vi "http.post.vi"(6 "specific headers in":cluster{"header":string, "Value":string}[](array[cluster]), 7 "Content Type":string="application/json", 8 "error in":errorcluster, 9 "Request body":string, 10 "Path":string, 11 "Nominal Client in":refnum<class "Nominal Client.lvclass">) -> (0 "error out":errorcluster, 2 "Response":string, 3 "Nominal Client out":refnum<class "Nominal Client.lvclass">)   [LabVIEW 2020, in "Nominal Client.lvclass"]
uses:
  Nominal Client.lvclass
  Nominal Client.lvclass/Nominal Client.ctl
  trace.calling_method.vi
  error.vi/859f8e04-e495-489b-b5b4-7ac163f56130.vi
  <vilib>/JDP Science/JDP Science Common Utilities/Trim Whitespace__JDP.vi
  <vilib>/AdvancedString/1D String Array to Delimited String.vi
  api_token.get.vi
  <vilib>/Utility/libraryn.llb/Get File Extension.vi
  log_file.write.vi
  <vilib>/JDP Science/JSONtext/Get all Object Items.vi
  <vilib>/Utility/error.llb/Error Cluster From Error Code.vi
  <vilib>/JDP Science/JSONtext/JSON text to Variant.vi
  <vilib>/JDP Science/JSONtext/LVClass Serializer/JSONtext LVClass Serializer.lvclass
  submodules/reqwest-labview/lv-src/reqwest/reqwest.lvclass
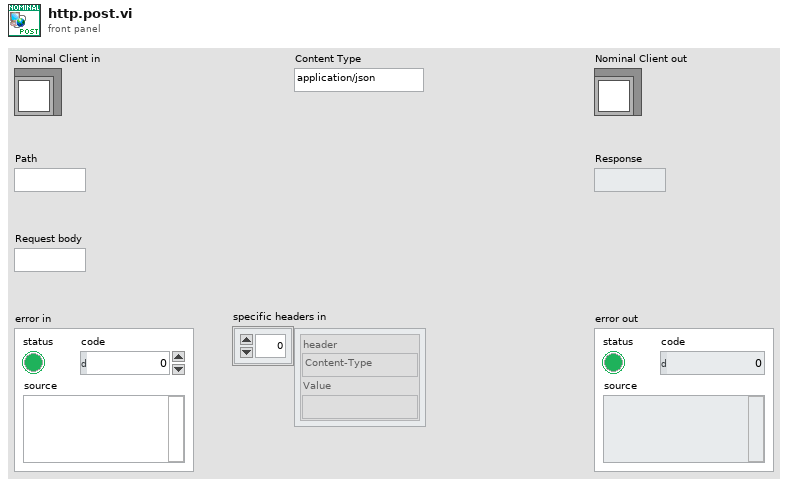
[diagram p1: front panel]
types:
  T1 = typedef "Nominal Client.lvclass/private_data.ctl" = cluster{"API Token":string, "workspace":refnum<class "workspace.lvclass">, "Available Workspaces":refnum<class "workspace.lvclass">[], "reqwest":refnum<class "reqwest.lvclass">}
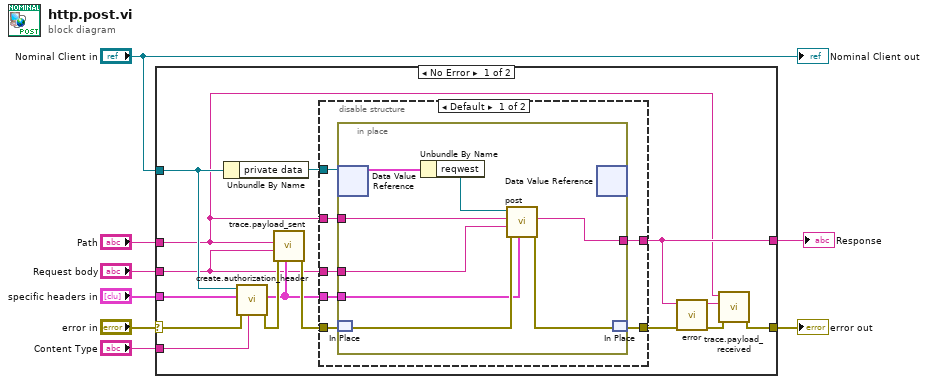
[diagram p0: block diagram]
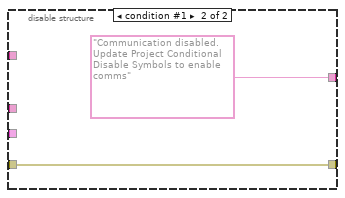
[diagram p2: hidden frame]
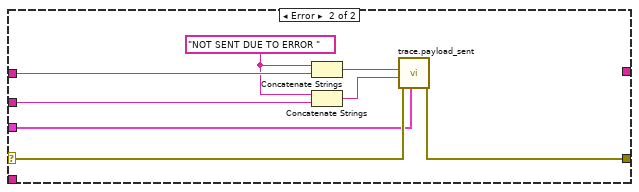
[diagram p3: hidden frame]
diagram:
  n1 = case shown="No Error" "error in" {
    selector: "error in" -> [w17 w43]
    tunnel: "Nominal Client in" -> [w21 _]
    tunnel: "specific headers in" -> [w18 w41]
    tunnel: "Request body" -> [w16 w45]
    tunnel: "Content Type" -> [w15 _]
    tunnel: [w14 _] -> w3
    tunnel: [w9 w42] -> w2
    tunnel: "Path" -> [w11 w47]
    frame No Error {
      n2 = Unbundle By Name(w21) -> ("private data"=w19:refnum<data-value>)
      n3 = call "create.authorization_header.vi"("Content Type"=w15, "error in"=w17, "specific headers in"=w18, "Nominal Client in"=w21) -> ("error out"=w23:errorcluster, "specific headers out"=w20:cluster{"header":string, "value":string}[])  [unwired: 5 in, 1 out]
      n4 = call "trace.payload_sent.vi"("Headers"=w20, "dataflow error in"=w23, "Request Body"=w16, "Path"=w11) -> ("dataflow error out"=w22:errorcluster)  [unwired: 7 in]
      n5 = disable-structure shown="Default" {
        disable-tunnel: w20 -> [w30 _]
        disable-tunnel: w19 -> [w29 _]
        disable-tunnel: w22 -> [w28 w40]
        disable-tunnel: w16 -> [w27 _]
        disable-tunnel: [w26 "Communication disabled. Update Project Conditional Disable Symbols to enable comms" ("REST Response")] -> w14
        disable-tunnel: [w25 w40] -> w12
        disable-tunnel: w11 -> [w24 _]
        frame condition #0 (active) {
          n6 = in-place {
            in-place-border: w30 -> [w34]
            in-place-border: [w36] -> w26
            in-place-border: w24 -> [w33]
            in-place-border: w27 -> [w35]
            n7 = in-place-dvr #1(w29) -> (w38:T1)  [unwired: 1 out]
            n8 = in-place-match #2(w28) -> (w37:errorcluster)
            n9 = Unbundle By Name(w38) -> ("reqwest"=w31:refnum<class "reqwest.lvclass">)
            n10 = call "post.vi"("request specific headers"=w34, "error in (no error)"=w37, "request body"=w35, "path"=w33, "reqwest in"=w31) -> ("error out"=w32:errorcluster, "response"=w36:string)  [unwired: 4 in, 1 out]
            n11 = in-place-dvr #1() -> ()  [unwired: 1 in, 2 out]
            n12 = in-place-match #2(w32) -> (w25:errorcluster)
          }
        }
        frame condition #1 {
        }
      }
      n13 = call "error.vi"("error in"=w12, "REST Response"=w14) -> ("error out"=w10:errorcluster, "Error Formatted Response"=w13:string)  [unwired: 8 in]
      n14 = call "trace.payload_received.vi"("dataflow error in"=w10, "Response"=w13, "Path"=w11) -> ("dataflow error out"=w9:errorcluster)  [unwired: 8 in]
    }
    frame Error {
      w46 = "NOT SENT DUE TO ERROR " ("string")
      n15 = Concatenate Strings(w46, w47) -> (w48:string)
      n16 = Concatenate Strings(w46, w45) -> (w44:string)
      n17 = call "trace.payload_sent.vi"("Headers"=w41, "dataflow error in"=w43, "Request Body"=w44, "Path"=w48) -> ("dataflow error out"=w42:errorcluster)  [unwired: 7 in]
    }
  }
  "error out" <- w2
  "Response" <- w3
  "Nominal Client out" <- "Nominal Client in"
